vi "Subscribe To Messages.vi"() -> ()   [LabVIEW 2018, in "Library.lvlib"]
uses:
  Library.lvlib
  <vilib>/Skyline/Message/HTTP Wrapper/Open (HTTP).vi
  <vilib>/Skyline/Message/HTTP Wrapper/NI Skyline Message HTTP.lvclass
  <vilib>/Skyline/Configuration/Configuration HTTP_class/NI Skyline Configuration HTTP.lvclass
  <vilib>/Skyline/Message/NI Skyline Message.lvclass
  <vilib>/Skyline/Configuration/Configuration_class/NI Skyline Configuration.lvclass
  <vilib>/Skyline/Configuration/Configuration HTTP_class/Open Configuration HTTP.vi
panel:
  out "error out":errorcluster
  out "Listbox":i32(listbox)
  out "Boolean":bool
  out "Publisher Loop Iteration":i32
  out "Message Received":string
  in  "stop":bool
  # "Overview: Demonstrates the use of the SystemLink Message functions. Use messages to send commands or configuration from one system or application to another. \n\nRequirements: SystemLink Server, SystemLink Cloud, or G Web Development Software\n\nInstructions:\n1. Ensure the local SystemLink Server is running or you have access to SystemLink Cloud\n2. Determine if this example is connecting to data available on SystemLink Server or SystemLink Cloud and use the appropriate version of Open Configuration VI \n3. Run this VI.\n4. Run webvi-examples\\CallSystemLinkDataServices\\Call SystemLink Data Services.gwebproject > BasicDataServices.gcomp > Read Write Messages.gviweb to generate messages from a WebVI"
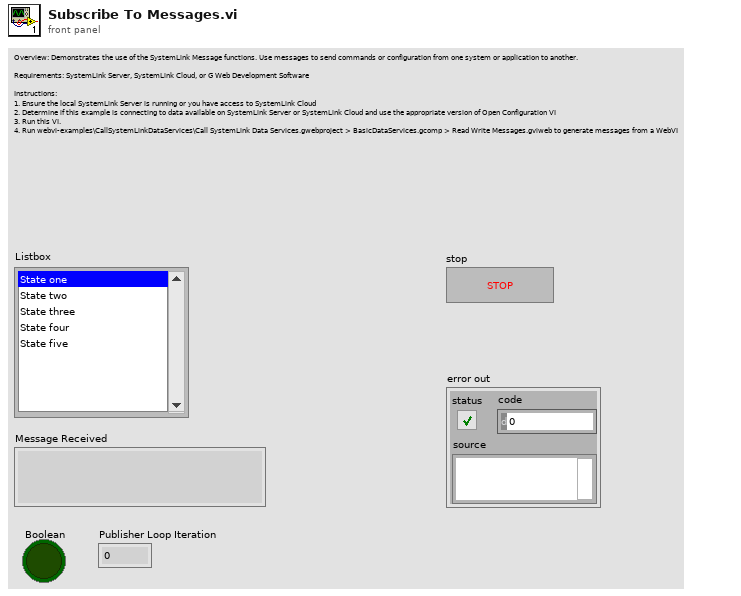
[diagram p1: front panel]
types:
  T1 = cluster{"Numeric":dbl, "Switch":bool, "State":i32, "String":string}
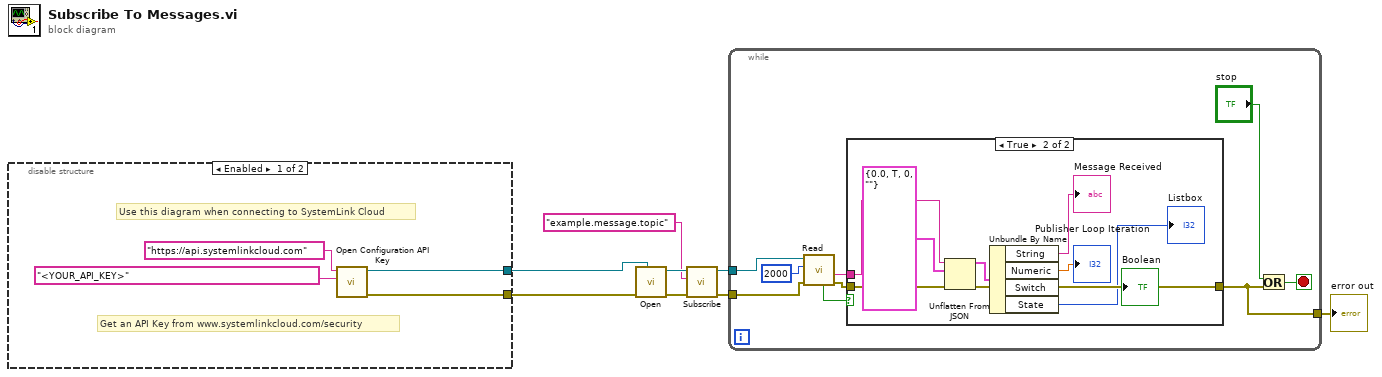
[diagram p0: block diagram]
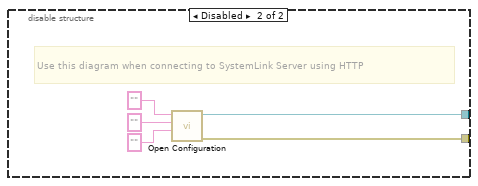
[diagram p2: hidden frame]
diagram:
  n1 = disable-structure shown="Enabled" {
    disable-tunnel: [w10 w17] -> w8
    disable-tunnel: [w9 w16] -> w7
    frame Enabled {
      # "Get an API Key from www.systemlinkcloud.com/security"
      # "Use this diagram when connecting to SystemLink Cloud"
      n2 = call <vilib>:"Open Configuration API Key.vi"("api key"="<YOUR_API_KEY>", "server url"="https://api.systemlinkcloud.com") -> ("error out"=w9:errorcluster, "configuration"=w10:refnum<class "NI Skyline Configuration HTTP.lvclass">)  [unwired: 8 in]
    }
    frame Disabled {
      # "Use this diagram when connecting to SystemLink Server using HTTP"
      n3 = call-poly <vilib>:"Open Configuration.vi"("password"="", "username"="", "server url"="") -> ("error out"=w16:errorcluster, "configuration"=w17:refnum<class "NI Skyline Configuration HTTP.lvclass">)  [unwired: 7 in]
    }
  }
  n4 = call-poly <vilib>:"Open.vi"("configuration"=w8, "error in (no error)"=w7) -> ("error out"=w4:errorcluster, "message session"=w6:refnum<class "NI Skyline Message HTTP.lvclass">)  [unwired: 8 in]
  n5 = call-dynamic "Subscribe.vi"("error in (no error)"=w4, "topic"="example.message.topic", "message session in"=w6) -> ("error out"=w2:errorcluster, "message session out"=w3:refnum<class "NI Skyline Message HTTP.lvclass">)  [unwired: 7 in]
  n6 = while {
    tunnel: w3 -> [w26]
    tunnel: w2 -> [w25]
    tunnel: [w18] -> w1
    stop <- w19 stop-if-true
    n7 = call-dynamic "Read.vi"("error in (no error)"=w25, "timeout milliseconds (100)"=2000, "sync message session in"=w26) -> ("error out"=w21:errorcluster, "message"=w22:string, "dequeue status"=w23:bool)  [unwired: 4 in, 2 out]
    n8 = case shown="True" w23 {
      tunnel: w22 -> [_ w36]
      tunnel: w21 -> [w27 w35]
      tunnel: [w27 w31] -> w18
      frame False {
        # "Timeout, do nothing"
      }
      frame True {
        n9 = Unflatten From JSON(JSON string=w36, type and defaults=T1 {"Numeric"=0.0, "Switch"=TRUE, "State"=0, "String"=""}, error in (no error)=w35) -> (value=w34:T1, error out=w31:errorcluster)  [unwired: 4 in]
        n10 = Unbundle By Name(w34) -> ("String"=→"Message Received":string, "Numeric"=→"Publisher Loop Iteration":dbl, "Switch"=→"Boolean":bool, "State"=→"Listbox":i32)
      }
    }
    n11 = Or(x="stop", y=w18) -> (x .or. y?=w19:bool)
  }
  "error out" <- w1
